vi "Update Value.vi"(6 "Time":dbl, 8 "error in (no error)":errorcluster, 11 "NumericCommandButton in":refnum<class "NumericCommandButton.lvclass">) -> (0 "error out":errorcluster, 1 "Update":bool, 2 "Value":variant, 3 "NumericCommandButton out":refnum<class "NumericCommandButton.lvclass">)   [LabVIEW 2025, in "VolatusGUIElements.lvlib" / "NumericCommandButton.lvclass"]
uses:
  NumericCommandButton.lvclass
  NumericCommandButton.lvclass/NumericCommandButton.ctl
  lv-vecto/Vecto/Channel DBL/Channel DBL.lvclass/Channel DBL.ctl
  lv-vecto/Vecto/Group DBL/Value by Index.vi
  lv-vecto/Vecto/Channel DBL/Channel DBL.lvclass
  VolatusGUIElements.lvlib
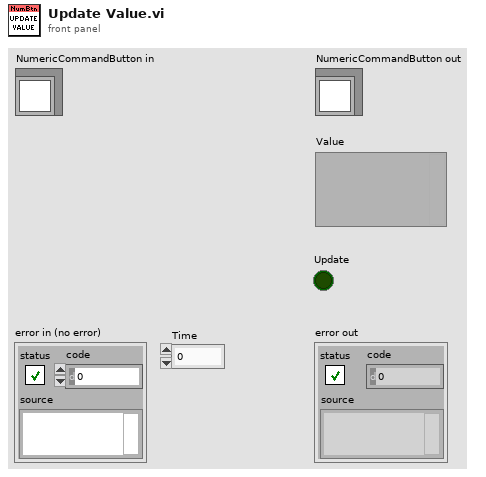
[diagram p1: front panel]
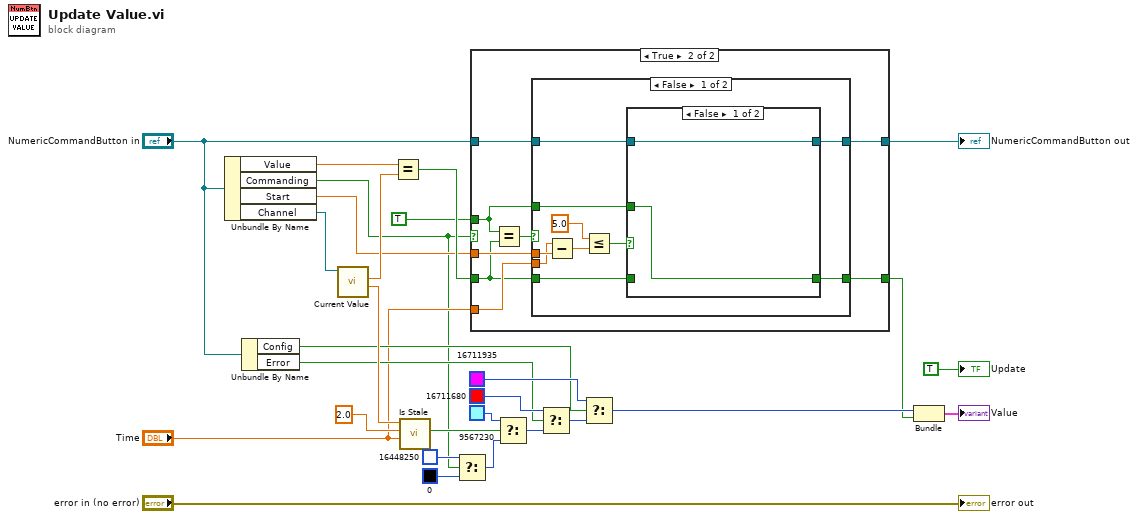
[diagram p0: block diagram]
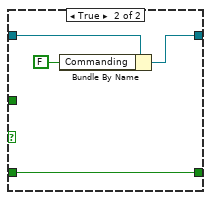
[diagram p3: hidden frame]
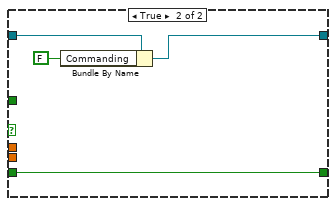
[diagram p4: hidden frame]
diagram:
  n1 = Unbundle By Name("NumericCommandButton in") -> ("Value"=w26:dbl, "Commanding"=w1:bool, "Start"=w7:dbl, "Channel"=w5:refnum<class "Channel DBL.lvclass">)
  n2 = Unbundle By Name("NumericCommandButton in") -> ("Config"=w13:bool, "Error"=w14:bool)
  n3 = call "Current Value.vi"("Channel in"=w5) -> ("Timestamp"=w16:dbl, "Scaled"=w25:dbl)  [unwired: 6 in, 3 out]
  n4 = Equal?(x=w26, y=w25) -> (x = y?=w9:bool)
  n5 = call "Is Stale.vi"("Time"="Time", "Staleness"=2.0, "Timestamp"=w16) -> ("Stale"=w23:bool)  [unwired: 8 in]
  n6 = Select(t=u32 16448250, s=w1, f=u32 0) -> (s? t:f=w4:u32)
  n7 = case shown="True" w1 {
    tunnel: w9 -> [w30 w35]
    tunnel: w7 -> [_ w38]
    tunnel: "Time" -> [_ w37]
    tunnel: TRUE -> [_ w31]
    tunnel: "NumericCommandButton in" -> [w29 w34]
    tunnel: [w29 w33] -> w27
    tunnel: [w30 w32] -> w11
    frame False {
    }
    frame True {
      n8 = Equal?(x=w31, y=w35) -> (x = y?=w36:bool)
      n9 = case shown="False" w36 {
        tunnel: w38 -> [w48 _]
        tunnel: w37 -> [w47 _]
        tunnel: w35 -> [w41 w55]
        tunnel: w34 -> [w43 w58]
        tunnel: [w42 w56] -> w33
        tunnel: [w39 w55] -> w32
        tunnel: w31 -> [w40 _]
        frame False {
          n10 = Subtract(x=w47, y=w48) -> (x-y=w46:dbl)
          n11 = Less Or Equal?(x=5.0, y=w46) -> (x <= y?=w44:bool)
          n12 = case shown="False" w44 {
            tunnel: w43 -> [w49 w54]
            tunnel: [w49 w52] -> w42
            tunnel: w41 -> [_ w51]
            tunnel: w40 -> [w50 _]
            tunnel: [w50 w51] -> w39
            frame False {
            }
            frame True {
              n13 = Bundle By Name(cluster=w54, "Commanding"=FALSE) -> (w52:refnum<class "NumericCommandButton.lvclass">)
            }
          }
        }
        frame True {
          n14 = Bundle By Name(cluster=w58, "Commanding"=FALSE) -> (w56:refnum<class "NumericCommandButton.lvclass">)
        }
      }
    }
  }
  "NumericCommandButton out" <- w27
  n15 = Select(t=u32 9567230, s=w23, f=w4) -> (s? t:f=w21:u32)
  n16 = Select(t=u32 16711680, s=w14, f=w21) -> (s? t:f=w19:u32)
  n17 = Select(t=u32 16711935, s=w13, f=w19) -> (s? t:f=w12:u32)
  n18 = Bundle(w12, w11) -> (→"Value":cluster{u32, bool})  [unwired: 1 in]
  "error out" <- "error in (no error)"
  "Update" <- TRUE ("Update")
